vi "RemoteVI Post At Cursor.vi"(0 "hWnd":u64, 5 "posts":cluster{"msg":u32, "wParam":u64, "lParam":i64}[](array[cluster]), 7 "lParam":i64, 11 "error in":errorcluster) -> (15 "error out":errorcluster)   [LabVIEW 2020, in "RemoteVI.lvlib"]
doc: "Posts a WM_MOUSEMOVE and then each message of posts to hWnd (the served panel) with lParam = the host cursor position in screen coordinates (RemoteVI Pack Point lParam.vi of GetCursorPos), each waiting until LabVIEW has handled it (RemoteVI Wait Input Handled.vi). Used by RemoteVI Plain Popup Click.vi once the clicked popup has been moved under the cursor: a popup ignores a click without the move before it (measured). An incoming error posts nothing."
uses:
  RemoteVI.lvlib
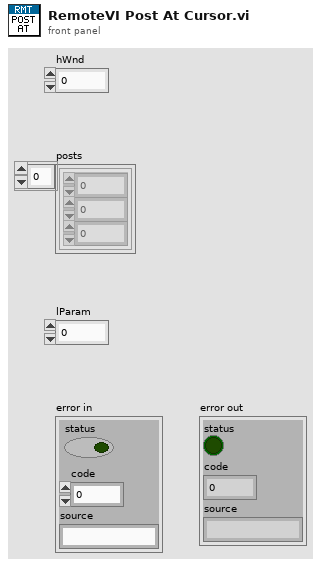
[diagram p1: front panel]
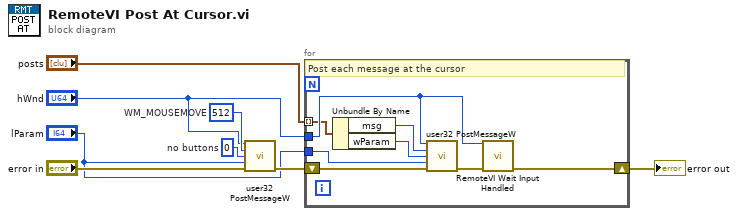
[diagram p0: block diagram]
diagram:
  w6 = u64 0  # no buttons
  w5 = u32 512  # WM_MOUSEMOVE
  n1 = call "user32 PostMessageW.vi"("hWnd"="hWnd", "Msg"=w5, "wParam"=w6, "lParam"="lParam", "error in (no error)"="error in") -> ("error out"=w7:errorcluster)  [unwired: 9 in, 1 out]
  n2 = for {
    tunnel: "posts" -> [w9] mode=indexing
    tunnel: "hWnd" -> [w10]
    tunnel: "lParam" -> [w11]
    shift-right: [w13] -> w8
    shift-left: w7 -> [w12]
    # "Post each message at the cursor"
    n3 = Unbundle By Name(w9) -> ("msg"=w14:u32, "wParam"=w15:u64)
    n4 = call "user32 PostMessageW.vi"("hWnd"=w10, "Msg"=w14, "wParam"=w15, "lParam"=w11, "error in (no error)"=w12) -> ("error out"=w16:errorcluster)  [unwired: 9 in, 1 out]
    n5 = call "RemoteVI Wait Input Handled.vi"("hWnd"=w10, "error in"=w16) -> ("error out"=w13:errorcluster)  [unwired: 13 in]
  }
  "error out" <- w8
